vi "tcp_test.vi"() -> ()   [LabVIEW 2020]
panel:
  out "error_out":errorcluster
  out "Numeric":i32
  out "data_out":dbl[](array[numeric]) format="%.6f"
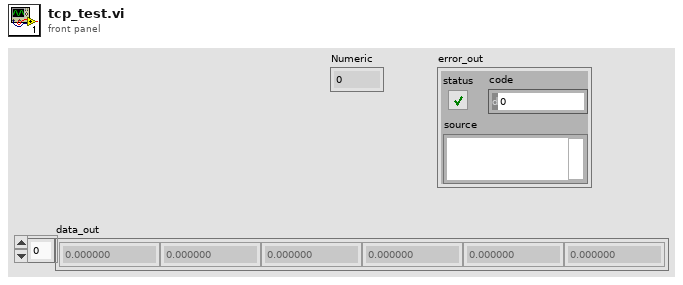
[diagram p1: front panel]
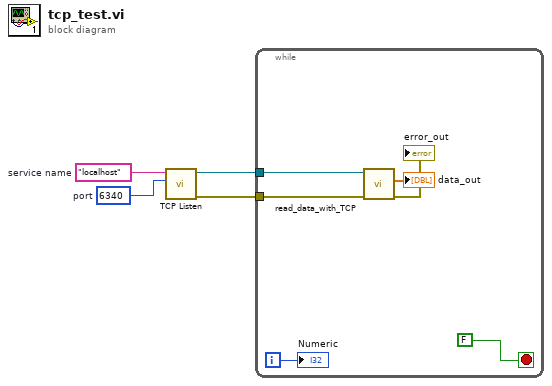
[diagram p0: block diagram]
diagram:
  w3 = u16 6340  # port
  w4 = "localhost"  # service name
  n1 = call <vilib>:"TCP Listen.vi"("port"=w3, "service name"=w4) -> ("error out"=w1:errorcluster, "connection ID"=w2:refnum<k5>)  [unwired: 5 in, 3 out]
  n2 = while {
    tunnel: w2 -> [w10]
    tunnel: w1 -> [w9]
    i -> [w7]
    stop <- FALSE stop-if-true
    n3 = call "read_data_with_TCP.vi"("error_in"=w9, "TCP_ref_in"=w10) -> ("error_out"=→"error_out":errorcluster, "data_out"=→"data_out":dbl[])  [unwired: 7 in, 1 out]
    "Numeric" <- w7
  }
